vi "CarWashTestcase.vi"(11 "error in":errorcluster) -> (4 "Wash Array":T1[](array[typedef]), 15 "error out":errorcluster)   [LabVIEW 2016, in "Car Wash Test.lvlib"]
uses:
  Car Wash Test.lvlib
  Controls/Wash Step Config.ctl
  <vilib>/addons/_JKI Toolkits/Caraya/classes/Test/Test.lvclass
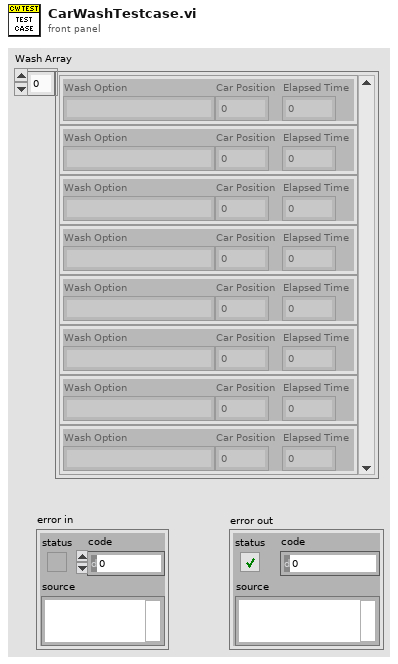
[diagram p1: front panel]
types:
  T1 = typedef "Car Wash Test.lvlib/Wash Step Config.ctl" = cluster{"Wash Option":string, "Car Position":i32, "Elapsed Time":dbl}
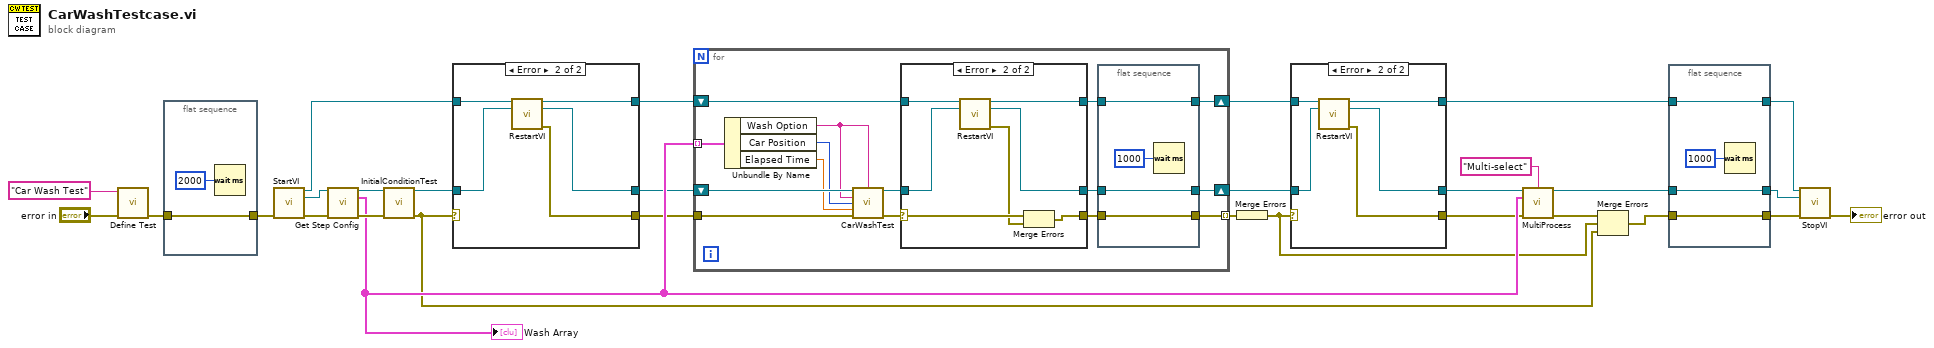
[diagram p0: block diagram]
diagram:
  n1 = call <vilib>:"Define Test.vi"("error in (no error)"="error in", "Label (VI Title)"="Car Wash Test" ("Label")) -> ("error out"=w18:errorcluster)  [unwired: 9 in]
  n2 = flat-sequence {
    tunnel: [w31] -> w17
    tunnel: w18 -> [w31]
    frame #0 {
      n3 = Wait (ms)(milliseconds to wait=u32 2000) -> ()  [unwired: 1 out]
    }
  }
  n4 = call "StartVI.vi"("error in"=w17) -> ("Application Ref out"=w4:refnum<vi>, "VI Reference"=w3:refnum<vi>, "error out"=w2:errorcluster)  [unwired: 12 in]
  n5 = call "Get Step Config.vi"("VI In"=w3, "error in"=w2) -> ("VI out"=w25:refnum<vi>, "Wash Array"=w23:T1[], "error out"=w24:errorcluster)  [unwired: 11 in]
  "Wash Array" <- w23
  n6 = call "InitialConditionTest.vi"("VI Reference In"=w25, "error in"=w24) -> ("VI Reference Out"=w10:refnum<vi>, "error out"=w7:errorcluster)  [unwired: 12 in]
  n7 = case shown="Error" w7 {
    selector: w7 -> [w34 _]
    tunnel: [w34 w40] -> w1
    tunnel: w10 -> [w35 w38]
    tunnel: [w35 w39] -> w9
    tunnel: [w33 w36] -> w11
    tunnel: w4 -> [w33 w37]
    frame No Error {
    }
    frame Error {
      n8 = call "RestartVI.vi"("Application Ref in"=w37, "VI in"=w38) -> ("Application Ref out"=w36:refnum<vi>, "VI out"=w39:refnum<vi>, "error out"=w40:errorcluster)  [unwired: 11 in]
    }
  }
  n9 = for {
    shift-right: [w44] -> w15
    shift-left: w9 -> [w54]
    tunnel: w23 -> [w53] mode=indexing
    tunnel: w1 -> [w55]
    tunnel: [w47] -> w26 mode=indexing
    shift-right: [w43] -> w16
    shift-left: w11 -> [w41]
    n10 = Unbundle By Name(w53) -> ("Wash Option"=w50:string, "Car Position"=w52:i32, "Elapsed Time"=w51:dbl)
    n11 = call "CarWashTest.vi"("VI Reference In"=w54, "Label"=w50, "Wash Option"=w50, "Car Position"=w52, "Elapsed Time"=w51, "error in"=w55) -> ("VI Reference Out"=w48:refnum<vi>, "error out"=w49:errorcluster)  [unwired: 8 in]
    n12 = case shown="Error" w49 {
      selector: w49 -> [w61 w69]
      tunnel: [w61 w68] -> w46
      tunnel: w48 -> [w62 w66]
      tunnel: [w62 w63] -> w45
      tunnel: [w60 w64] -> w42
      tunnel: w41 -> [w60 w65]
      frame No Error {
      }
      frame Error {
        n13 = call "RestartVI.vi"("Application Ref in"=w65, "VI in"=w66) -> ("Application Ref out"=w64:refnum<vi>, "VI out"=w63:refnum<vi>, "error out"=w67:errorcluster)  [unwired: 11 in]
        n14 = Merge Errors(w69, w67) -> (w68:errorcluster)
      }
    }
    n15 = flat-sequence {
      tunnel: [w59] -> w47
      tunnel: w46 -> [w59]
      tunnel: w45 -> [w58]
      tunnel: [w58] -> w44
      tunnel: [w57] -> w43
      tunnel: w42 -> [w57]
      frame #0 {
        n16 = Wait (ms)(milliseconds to wait=u32 1000) -> ()  [unwired: 1 out]
      }
    }
  }
  n17 = Merge Errors(w26) -> (w6:errorcluster)
  n18 = case shown="Error" w6 {
    selector: w6 -> [w71 _]
    tunnel: [w71 w77] -> w12
    tunnel: w15 -> [w72 w75]
    tunnel: [w72 w76] -> w14
    tunnel: [w70 w73] -> w13
    tunnel: w16 -> [w70 w74]
    frame No Error {
    }
    frame Error {
      n19 = call "RestartVI.vi"("Application Ref in"=w74, "VI in"=w75) -> ("Application Ref out"=w73:refnum<vi>, "VI out"=w76:refnum<vi>, "error out"=w77:errorcluster)  [unwired: 11 in]
    }
  }
  n20 = call "MultiProcess.vi"("VI Reference In"=w14, "Label"="Multi-select", "Wash Array"=w23, "error in"=w12) -> ("VI Reference Out"=w22:refnum<vi>, "error out"=w5:errorcluster)  [unwired: 10 in]
  n21 = Merge Errors(w5, w6, w7) -> (w8:errorcluster)
  n22 = flat-sequence {
    tunnel: [w81] -> w19
    tunnel: w8 -> [w81]
    tunnel: w22 -> [w78]
    tunnel: [w80] -> w20
    tunnel: w13 -> [w80]
    tunnel: [w78] -> w21
    frame #0 {
      n23 = Wait (ms)(milliseconds to wait=u32 1000) -> ()  [unwired: 1 out]
    }
  }
  n24 = call "StopVI.vi"("Application Ref in"=w20, "VI in"=w21, "error in (no error)"=w19) -> ("error out"=→"error out":errorcluster)  [unwired: 12 in]
